vi "move right click menu.vi"(8 "error in":errorcluster, 10 "Point32":T1, 11 "VI":refnum<vi>) -> (0 "error out":errorcluster)   [LabVIEW 2013, in "control module editor.lvclass"]
uses:
  control module editor.lvclass
  <vilib>/Utility/miscctls.llb/LVPoint32TypeDef.ctl
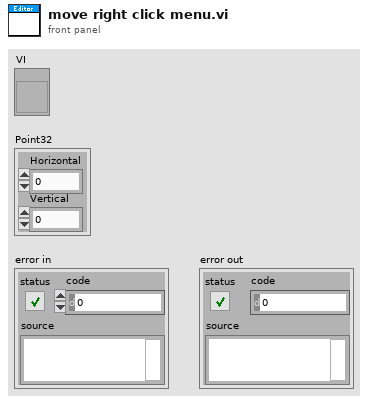
[diagram p1: front panel]
types:
  T1 = typedef "LVPoint32TypeDef.ctl" = cluster{"Horizontal":i32, "Vertical":i32}
  T2 = typedef "LVAllMonitorsDisplayTypeDef.ctl" = cluster{"Bounds":cluster{"Left":i16, "Top":i16, "Right":i16, "Bottom":i16}, "Depth":i16}[]
  T3 = typedef "LVRectTypeDef.ctl" = cluster{"Left":i16, "Top":i16, "Right":i16, "Bottom":i16}
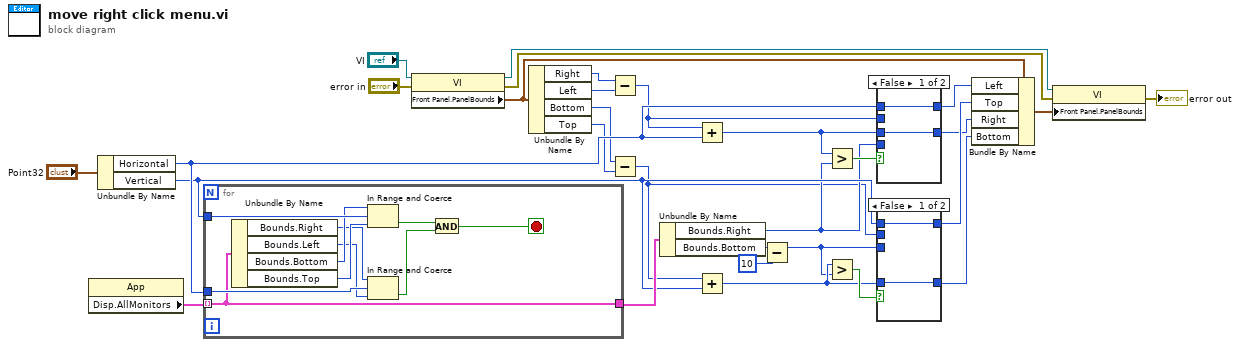
[diagram p0: block diagram]
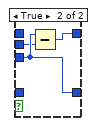
[diagram p2: hidden frame]
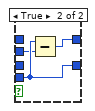
[diagram p3: hidden frame]
diagram:
  n1 = property class="App"() -> ("Disp.AllMonitors"=w25:T2)  [unwired: 2 in, 2 out]
  n2 = Unbundle By Name("Point32") -> ("Horizontal"=w21:i32, "Vertical"=w20:i32)
  n3 = for {
    tunnel: w25 -> [w37] mode=indexing
    tunnel: w21 -> [w40]
    tunnel: w20 -> [w35]
    tunnel: [w37] -> w24
    stop <- w36 stop-if-true
    n4 = Unbundle By Name(w37) -> ("Bounds.Right"=w31:i16, "Bounds.Left"=w32:i16, "Bounds.Bottom"=w33:i16, "Bounds.Top"=w34:i16)
    n5 = In Range and Coerce(upper limit=w33, x=w35, lower limit=w34) -> (In Range?=w38:bool)  [unwired: 1 out]
    n6 = In Range and Coerce(upper limit=w31, x=w40, lower limit=w32) -> (In Range?=w39:bool)  [unwired: 1 out]
    n7 = And(x=w38, y=w39) -> (x .and. y?=w36:bool)
  }
  n8 = property class="VI"(reference="VI", error in="error in") -> (reference out=w3:refnum<vi>, error out=w27:errorcluster, "Front Panel.PanelBounds"=w5:T3)
  n9 = Unbundle By Name(w5) -> ("Right"=w8:i16, "Left"=w7:i16, "Bottom"=w11:i16, "Top"=w10:i16)
  n10 = Subtract(x=w8, y=w7) -> (x-y=w6:i16)
  n11 = Subtract(x=w11, y=w10) -> (x-y=w9:i16)
  n12 = Unbundle By Name(w24) -> ("Bounds.Right"=w12:i16, "Bounds.Bottom"=w13:i16)
  n13 = Add(x=w6, y=w21) -> (x+y=w16:i32)
  n14 = Add(x=w9, y=w20) -> (x+y=w15:i32)
  n15 = Subtract(x=w13, y=i16 10) -> (x-y=w2:i16)
  n16 = Greater?(x=w16, y=w12) -> (0:w23:bool)
  n17 = Greater?(x=w15, y=w2) -> (0:w19:bool)
  n18 = case shown="False" w23 {
    tunnel: [w42 w43] -> w22
    tunnel: w21 -> [w42 _]
    tunnel: [w41 w45] -> w17
    tunnel: w16 -> [w41 _]
    tunnel: w12 -> [_ w45]
    tunnel: w6 -> [_ w44]
    frame False {
    }
    frame True {
      n19 = Subtract(x=w45, y=w44) -> (x-y=w43:i16)
    }
  }
  n20 = case shown="False" w19 {
    tunnel: [w47 w50] -> w18
    tunnel: w20 -> [w47 _]
    tunnel: w15 -> [w46 _]
    tunnel: [w46 w49] -> w14
    tunnel: w2 -> [_ w49]
    tunnel: w9 -> [_ w48]
    frame False {
    }
    frame True {
      n21 = Subtract(x=w49, y=w48) -> (x-y=w50:i16)
    }
  }
  n22 = Bundle By Name(cluster=w5, "Left"=w22, "Top"=w18, "Right"=w17, "Bottom"=w14) -> (w29:T3)
  n23 = property class="VI"(reference=w3, error in=w27, "Front Panel.PanelBounds"=w29) -> (error out=→"error out":errorcluster)  [unwired: 1 out]
